vi "VIH Dialog - VI Terminals - Build Control Tree.vi"(6 "Ctrl Attributes":T1[](array[typedef]), 8 "error in":errorcluster, 9 "Parent tag":string, 10 "Tree Refnum":refnum<vi>, 11 "Ctrl Refnums":refnum<vi>[](array[refnum])) -> (0 "error out":errorcluster, 1 "Control Rules":T3[](array[typedef]), 2 "Controls Info":T2(array[cluster]), 3 "dup Ctrl Refnums":refnum<vi>[](array[refnum]))   [LabVIEW 2014]
doc: "::: VI Helpeks :::\nCopyright (c) 2000-2026 Konstantin Shifershteyn. All rights reserved."
uses:
  _VIH HelpGen.llb/VIH HelpGen Typedef - Cluster - Control Rule.ctl
  _VIH HelpGen.llb/VIH HelpGen Typedef - Enum - Description Mode.ctl
  _VIH HelpGen.llb/VIH HelpGen Typedef - Enum - Default,Enable,Disable.ctl
  _VIH HelpGen.llb/VIH HelpGen Typedef - Cluster - Enum Value Info.ctl
  _VIH HelpGen.llb/VIH HelpGen Typedef - Control Terminal Attributes Cluster.ctl
panel:
  # "VI Helpeks\nCopyright (c) 2012-2026 Konstantin Shifershteyn"
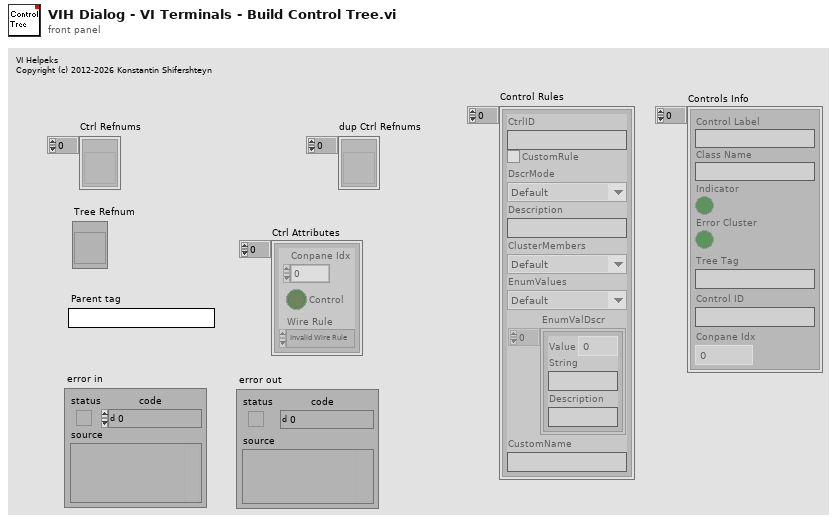
[diagram p1: front panel]
types:
  T1 = typedef "VIH HelpGen Typedef - Control Terminal Attributes Cluster.ctl" = cluster{"Conpane Idx":i32, "Control":bool, "Wire Rule":enum16{"Invalid Wire Rule", "Required", "Recommended", "Optional", "Dynamic Dispatch"}}
  T2 = cluster{"Control Label":string, "Class Name":string, "Indicator":bool, "Error Cluster":bool, "Tree Tag":string, "Control ID":string, "Conpane Idx":i32}[]
  T3 = typedef "VIH HelpGen Typedef - Cluster - Control Rule.ctl" = cluster{"CtrlID":string, "CustomRule":bool, "DscrMode":T4, "Description":string, "ClusterMembers":T5, "EnumValues":T5, "EnumValDscr":T6[], "CustomName":string}
  T4 = typedef "VIH HelpGen Typedef - Enum - Description Mode.ctl" = enum16{"Default", "Description", "Description1", "Description2", "Custom", "None"}
  T5 = typedef "VIH HelpGen Typedef - Enum - Default,Enable,Disable.ctl" = enum16{"Default", "Enable", "Disable"}
  T6 = typedef "VIH HelpGen Typedef - Cluster - Enum Value Info.ctl" = cluster{"Value":ext, "String":string, "Description":string}
  T7 = enum16{"nop", "Init", "get index", "get symbols"}
  T8 = cluster{"Label":string, "Class Name":string, "Indicator":bool, "Error Cluster":bool, "Edit Tree Items:Add Item":string, "Control Tag":string, "Conpane Idx":i32}
  T9 = typedef "imagedata.ctl" = cluster{"image type":i32, "image depth":i32, "image":u8[], "mask":u8[], "colors":u32[], "Rectangle":cluster{"left":i16, "top":i16, "right":i16, "bottom":i16}}
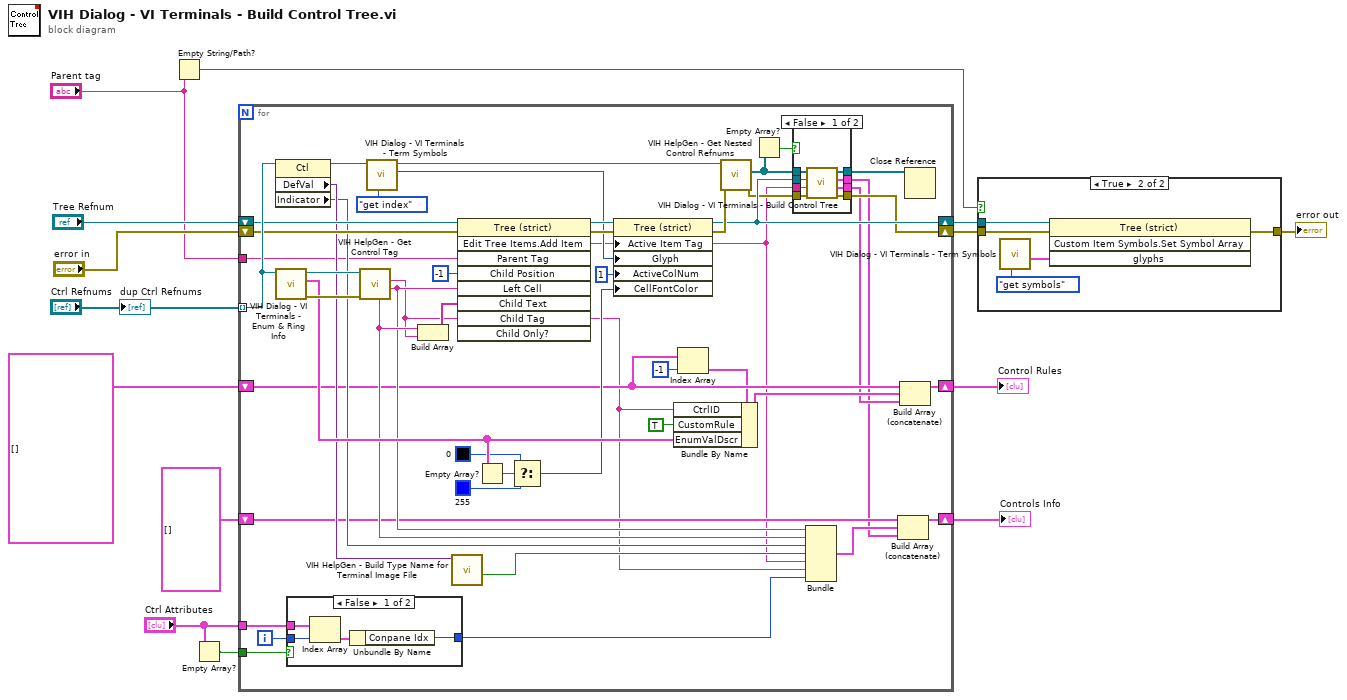
[diagram p0: block diagram]
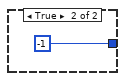
[diagram p3: hidden frame]
diagram:
  n1 = Empty String/Path?(string/path="Parent tag") -> (empty?=w8:bool)
  n2 = Empty Array?(array="Ctrl Attributes") -> (empty?=w1:bool)
  n3 = for {
    tunnel: "Ctrl Refnums" -> [w59] mode=indexing
    shift-right: [w35] -> w12
    shift-left: "Tree Refnum" -> [w55]
    shift-right: [w31] -> w10
    shift-left: "error in" -> [w48]
    tunnel: "Parent tag" -> [w39]
    shift-right: [w30] -> w6
    shift-left: T3[] [] ("Control Rules") -> [w27]
    shift-right: [w23] -> w3
    shift-left: T2 [] ("Controls Info") -> [w24]
    tunnel: "Ctrl Attributes" -> [w18]
    tunnel: w1 -> [w16]
    i -> [w17]
    n4 = property class="Ctl"(reference=w59) -> (reference out=w42:refnum<vi>, "DefVal"=w47:variant, "Indicator"=w45:bool)  [unwired: 1 in, 1 out]
    n5 = call "VIH Dialog - VI Terminals - Enum & Ring Info.vi"("Ctl Refnum"=w59) -> ("error out"=w58:errorcluster, "EnumValDscr"=w52:T6[], "dup Ctl Refnum"=w60:refnum<vi>)  [unwired: 8 in]
    n6 = case shown="False" w16 {
      tunnel: w18 -> [w67 _]
      tunnel: w17 -> [w66 _]
      tunnel: [w64 -1 ("Conpane Idx")] -> w15
      frame False {
        n7 = Index Array(array=w67, index=w66) -> (element=w65:T1)
        n8 = Unbundle By Name(w65) -> ("Conpane Idx"=w64:i32)
      }
      frame True {
      }
    }
    n9 = call "VIH HelpGen - Get Control Tag.vi"("error in"=w58, "Ctl Refnum"=w60) -> ("Label"=w43:string, "Control Tag"=w19:string, "Class Name"=w46:string)  [unwired: 4 in, 3 out]
    n10 = call "VIH Dialog - VI Terminals - Term Symbols.vi"("cmd (nop)"=T7."get index", "Ctl Refnum"=w42) -> ("Symbol Index"=w41:i32, "dup Ctl Refnum"=w38:refnum<vi>)  [unwired: 6 in, 2 out]
    n11 = Build Array(w46, w19) -> (w62:string[])
    n12 = call "VIH HelpGen - Build Type Name for Terminal Image File.vi"("variant"=w47) -> ("Error Cluster"=w44:bool)  [unwired: 9 in, 1 out]
    n13 = invoke on="Invoke Node" class="Tree (strict)" method="Edit Tree Items.Add Item"(reference=w55, error in=w48, "Parent Tag"=w39, "Child Position"=-1, "Left Cell"=w43, "Child Text"=w62, "Child Tag"=w19) -> (reference out=w56:refnum<vi>, error out=w61:errorcluster, "Edit Tree Items:Add Item"=w20:string)  [unwired: 2 in, 6 out]
    n14 = Empty Array?(array=w52) -> (empty?=w53:bool)
    n15 = Select(t=u32 0, s=w53, f=u32 255) -> (s? t:f=w49:u32)
    n16 = property on="Property Node" class="Tree (strict)"(reference=w56, error in=w61, "Active Item Tag"=w20, "Glyph"=w41, "ActiveColNum"=1 ("Active Cell:Active Column Number"), "CellFontColor"=w49) -> (reference out=w35:refnum<vi>, error out=w37:errorcluster)
    n17 = Index Array(array=w27, index=-1) -> (element=w26:T3)
    n18 = Bundle By Name(cluster=w26, "CtrlID"=w19, "CustomRule"=TRUE, "EnumValDscr"=w52) -> (w29:T3)
    n19 = call "VIH HelpGen - Get Nested Control Refnums.vi"("error in"=w37, "Ctl Refnum"=w38) -> ("error out"=w34:errorcluster, "Ctl Refnums"=w36:refnum<vi>[])  [unwired: 7 in, 1 out]
    n20 = Empty Array?(array=w36) -> (empty?=w33:bool)
    n21 = case shown="False" w33 {
      tunnel: w36 -> [w76 w78]
      tunnel: w35 -> [w75 _]
      tunnel: w20 -> [w74 _]
      tunnel: w34 -> [w73 w77]
      tunnel: [w72 w78] -> w32
      tunnel: [w71 w77] -> w31
      tunnel: [w70 _] -> w25
      tunnel: [w69 _] -> w21
      frame False {
        n22 = call "VIH Dialog - VI Terminals - Build Control Tree.vi"("error in"=w73, "Parent tag"=w74, "Tree Refnum"=w75, "Ctrl Refnums"=w76) -> ("error out"=w71:errorcluster, "Control Rules"=w70:T3[], "Controls Info"=w69:T2, "dup Ctrl Refnums"=w72:refnum<vi>[])  [unwired: 4 in]
      }
      frame True {
      }
    }
    n23 = Bundle("Label"=w43, "Class Name"=w46, "Indicator"=w45, "Error Cluster"=w44, "Edit Tree Items:Add Item"=w20, "Control Tag"=w19, "Conpane Idx"=w15) -> (w22:T8)  [unwired: 1 in]
    n24 = Build Array (concatenate)(w24, w22, w21) -> (w23:T2)
    n25 = Build Array (concatenate)(w27, w29, w25) -> (w30:T3[])
    n26 = Close Reference(reference=w32) -> ()  [unwired: 1 in, 1 out]
  }
  "Control Rules" <- w6
  "Controls Info" <- w3
  n27 = case shown="True" w8 {
    tunnel: w12 -> [_ w84]
    tunnel: w10 -> [w79 w83]
    tunnel: [w79 w82] -> w9
    frame False {
    }
    frame True {
      n28 = call "VIH Dialog - VI Terminals - Term Symbols.vi"("cmd (nop)"=T7."get symbols") -> ("Symbols"=w80:T9[])  [unwired: 7 in, 3 out]
      n29 = invoke on="Invoke Node" class="Tree (strict)" method="Custom Item Symbols.Set Symbol Array"(reference=w84, error in=w83, "glyphs"=w80) -> (error out=w82:errorcluster)  [unwired: 1 in, 3 out]
    }
  }
  "error out" <- w9
  "dup Ctrl Refnums" <- "Ctrl Refnums"
